vi "Turn to Tag.vi"(8 "error in (no error)":errorcluster, 9 "Command Info In":T1, 11 "Synchronization":enum16{"Start", "Wait"}(ring)=enum."Wait") -> (0 "error out":errorcluster, 1 "Command Info Out":T1)   [LabVIEW 2025]
doc: "Drive command composition: stop and acquire a fresh Limelight 3a AprilTag heading; submit Turn to Angle only when valid. Synchronization defaults to Wait. A missing/stale tag skips the turn."
uses:
  <vilib>/Rock Robotics/WPI/Framework/Command Status Info.ctl
  <vilib>/Rock Robotics/WPI/Framework/Completion Status.ctl
  <vilib>/Rock Robotics/WPI/Framework/Completion Notifier.ctl
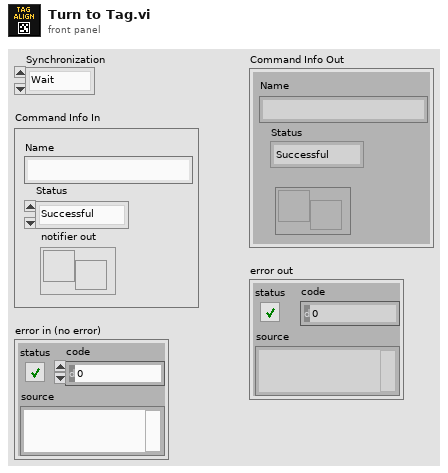
[diagram p1: front panel]
types:
  T1 = typedef "Command Status Info.ctl" = cluster{"Name":string, "Status":T2, "notifier out":T3}
  T2 = typedef "Completion Status.ctl" = enum16{"Successful", "Aborted", "Incomplete"}
  T3 = typedef "Completion Notifier.ctl" = refnum<notifier>
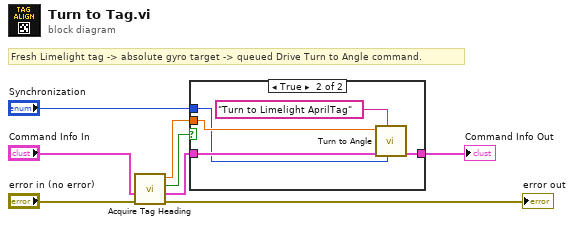
[diagram p0: block diagram]
diagram:
  # "Fresh Limelight tag -> absolute gyro target -> queued Drive Turn to Angle command."
  n1 = call "Acquire Tag Heading.vi"("error in (no error)"="error in (no error)", "Command Info In"="Command Info In") -> ("error out"=→"error out":errorcluster, "Command Info Out"=w2:T1, "Acquired"=w7:bool, "Target Heading"=w6:dbl)  [unwired: 6 in]
  n2 = case shown="True" w7 {
    tunnel: w6 -> [_ w13]
    tunnel: "Synchronization" -> [_ w11]
    tunnel: [w9 w10] -> w3
    tunnel: w2 -> [w9 w12]
    frame False {
    }
    frame True {
      n3 = call "Turn to Angle.vi"("Synchronization"=w11, "Description"="Turn to Limelight AprilTag", "Command Info In"=w12, "Angle"=w13) -> ("Command Info Out"=w10:T1)  [unwired: 7 in]
    }
  }
  "Command Info Out" <- w3
